vi "XMLCreate.vi"(8 "Error In":errorcluster, 11 "DOM document in":refnum<k20>) -> (0 "Error Out":errorcluster, 1 "server endpoint URL":string, 2 "OPC UA server refnum out":refnum<k21>, 3 "DOM document out":refnum<k20>)   [LabVIEW 2014, in "OPCUA XML(dev).lvlib"]
uses:
  OPCUA XML(dev).lvlib
  <resource>/objmgr/DOMUserDefRef.rc
  <vilib>/xml/NI_XML.lvlib
  <vilib>/OPCUA/NI OPC UA Server.lvlib
  <vilib>/xml/Close Reference(Node).vi
  <vilib>/xml/Close Reference(NdList).vi
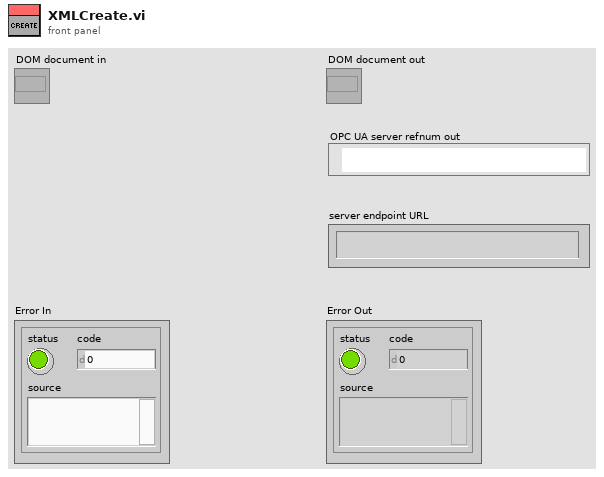
[diagram p1: front panel]
types:
  T1 = typedef "supported security policies.ctl" = cluster{"None":bool, "Sign with Basic128Rsa125":bool, "Sign and Encrypt with Basic128Rsa125":bool, "Sign with Basic256":bool, "Sign and Encrypt with Basic256":bool}
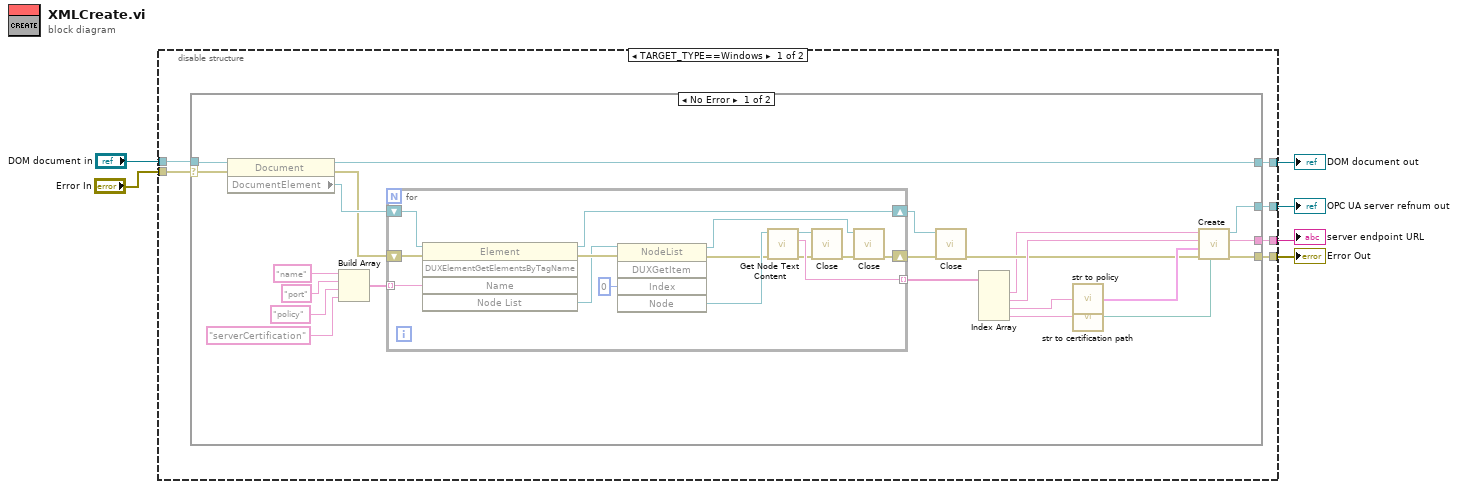
[diagram p0: block diagram]
diagram:
  n1 = disable-structure shown="TARGET_TYPE==Windows" {
    disable-tunnel: [w12 w54] -> w6
    disable-tunnel: "Error In" -> [w11 w54]
    disable-tunnel: "DOM document in" -> [w10 w53]
    disable-tunnel: [w9 w53] -> w3
    disable-tunnel: [w8 _] -> w2
    disable-tunnel: [w7 _] -> w1
    frame condition #0 {
      n2 = case shown="No Error" w11 {
        selector: w11 -> [w35 w52]
        tunnel: [w19 w52] -> w12
        tunnel: w10 -> [w34 w51]
        tunnel: [w33 w51] -> w9
        tunnel: [w21 _] -> w7
        tunnel: [w20 _] -> w8
        frame No Error {
          n3 = property class="Document"(reference=w34, error in=w35) -> (reference out=w33:refnum<k20>, error out=w31:errorcluster, "DocumentElement"=w32:refnum<k20>)
          n4 = Build Array("name" ("Name"), "port" ("Name"), "policy" ("Name"), "serverCertification" ("Name")) -> (w26:string[])
          n5 = for {
            tunnel: w26 -> [w48] mode=indexing
            tunnel: [w43] -> w25 mode=indexing
            shift-right: [w38] -> w18
            shift-left: w31 -> [w49]
            shift-right: [w37] -> w17
            shift-left: w32 -> [w50]
            n6 = invoke class="Element" method="DUXElementGetElementsByTagName"(reference=w50, error in=w49, "Name"=w48) -> (reference out=w37:refnum<k20>, error out=w46:errorcluster, "Node List"=w45:refnum<k20>)  [unwired: 2 in, 2 out]
            n7 = invoke class="NodeList" method="DUXGetItem"(reference=w45, error in=w46, "Index"=0) -> (reference out=w39:refnum<k20>, error out=w36:errorcluster, "Node"=w44:refnum<k20>)  [unwired: 2 in, 2 out]
            n8 = call <vilib>:"Get Node Text Content.vi"("error in (no error)"=w36, "node in"=w44) -> ("error out"=w42:errorcluster, "node text"=w43:string, "node out"=w41:refnum<k20>)  [unwired: 7 out]
            n9 = call-poly <vilib>:"Close.vi"("error in (no error)"=w42, "node"=w41) -> ("error out"=w40:errorcluster)  [unwired: 7 out]
            n10 = call-poly <vilib>:"Close.vi"("error in (no error)"=w40, "node list"=w39) -> ("error out"=w38:errorcluster)  [unwired: 7 out]
          }
          n11 = call-poly <vilib>:"Close.vi"("error in (no error)"=w18, "node"=w17) -> ("error out"=w16:errorcluster)  [unwired: 7 out]
          n12 = Index Array(array=w25) -> (element #1=w15:string, element #2=w24:string, element #3=w23:string, element #4=w13:string)  [unwired: 4 in]
          n13 = call "str to policy.vi"("String"=w23) -> ("supported security policies (None)"=w22:T1)  [unwired: 6 in]
          n14 = call "str to certification path.vi"("node text"=w13) -> ("File Path Control"=w14:path)  [unwired: 4 in]
          n15 = call <vilib>:"Create.vi"("server certificate file"=w14, "error in (no error)"=w16, "supported security policies (None)"=w22, "TCP port (49580)"=w24, "OPC UA server name"=w15) -> ("error out"=w19:errorcluster, "server endpoint URL"=w20:string, "OPC UA server refnum out"=w21:refnum<k21>)  [unwired: 4 in]
        }
        frame Error {
        }
      }
    }
    frame condition #1 (active) {
    }
  }
  "Error Out" <- w6
  "DOM document out" <- w3
  "OPC UA server refnum out" <- w1
  "server endpoint URL" <- w2
